vi "test_TwoSessTwoPinTwoInstrTwoSiteReservation_CallNiFgenGetConnections1Pin1Connection_ReturnsOneConnection.vi"(8 "error in":errorcluster) -> (0 "error out":errorcluster, 2 "result":string, 3 "pass":bool)   [LabVIEW 2021, in "MeasurementServerTests.lvlib"]
uses:
  MeasurementServerTests.lvlib
  Runtime/Clients/Session Management V1/Session Reservation/Connection.ctl
  Runtime/Sessions/niFGEN/Connection with Session.ctl
  03fc85e1-696b-4ece-a78b-f41470766ac0.vi
  ee969218-a503-4951-836c-6bb19e4d29f5.vi
  <vilib>/AdvancedString/1D String Array to Delimited String.vi
  ee969218-a503-4951-836c-6bb19e4d29f5.vi/94283ac5-2298-4b3a-b57d-7be67da3787d.vi
  ee969218-a503-4951-836c-6bb19e4d29f5.vi/f7d9c9cb-0251-4d67-81cb-70e1b0e8b69f.vi
  Runtime/Sessions/niFGEN/Get Connections - 1Pin 1Conn.vi
  <vilib>/JDP Science/JSONtext/Variant to JSON Text.vi
  <vilib>/JDP Science/JSONtext/LVClass Serializer/JSONtext LVClass Serializer.lvclass
  Runtime/Clients/Session Management V1/Session Reservation/Session Reservation.lvclass
  Runtime/Sessions/niFGEN/NI Session Management niFGEN.lvlib
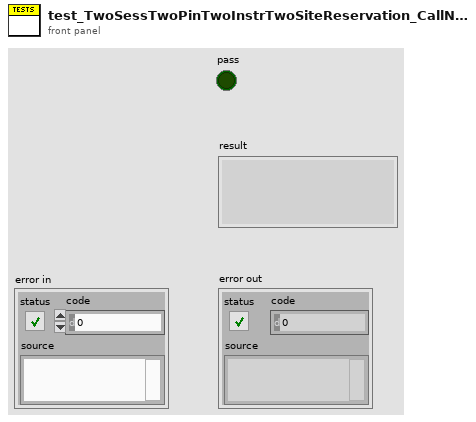
[diagram p1: front panel]
types:
  T1 = typedef "NI Session Management niFGEN.lvlib/Connection with Session.ctl" = cluster{"connection":T2, "session":refnum<k15>}
  T2 = typedef "NI Session Management V1 Client.lvlib/Session Reservation.lvclass/Connection.ctl" = cluster{"pin or relay name":string, "site":i32, "instrument type id":string, "channel":string}
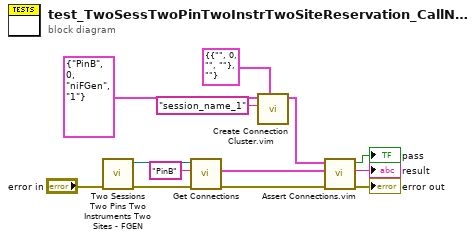
[diagram p0: block diagram]
diagram:
  n1 = call "Two Sessions Two Pins Two Instruments Two Sites - FGEN.vi"("error in"="error in") -> ("error out"=w5:errorcluster, "session reservation out"=w6:refnum<class "Session Reservation.lvclass">)  [unwired: 9 in]
  n2 = call-poly "Get Connections.vi"("error in"=w5, "pin or relay name"="PinB", "session reservation in"=w6) -> ("error out"=w4:errorcluster, "connection"=w1:T1)  [unwired: 6 in, 1 out]
  n3 = call "Create Connection Cluster.vim"("connection type"=T1 {"connection"={"pin or relay name"="", "site"=0, "instrument type id"="", "channel"=""}, "session"=""} ("niDCPower connection"), "session in"="session_name_1", "hardware independent connection in"=T2 {"pin or relay name"="PinB", "site"=0, "instrument type id"="niFGen", "channel"="1"} ("connection")) -> ("connection out"=w2:T1)  [unwired: 8 in]
  n4 = call "Assert Connections.vim"("error in"=w4, "actual connections"=w1, "expected connections"=w2) -> ("error out"=→"error out":errorcluster, "result"=→"result":string, "pass"=→"pass":bool)  [unwired: 6 in]
